vi "Reinitialize.vi"(8 "error in (no error)":errorcluster, 11 "ProPar in":refnum<class "PL Bronkhorst ProPar.lvclass">) -> (0 "error out":errorcluster, 3 "ProPar out":refnum<class "PL Bronkhorst ProPar.lvclass">)   [LabVIEW 2015, in "PL Bronkhorst ProPar.lvclass"]
doc: "Reinitializes connection to device based on previously specified settings."
uses:
  PL Bronkhorst ProPar.lvclass
  PL Bronkhorst ProPar.lvclass/PL Bronkhorst ProPar.ctl
  <vilib>/Instr/_visa.llb/VISA Configure Serial Port (Instr).vi
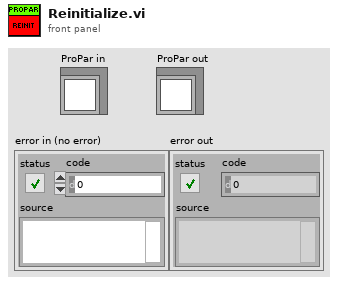
[diagram p1: front panel]
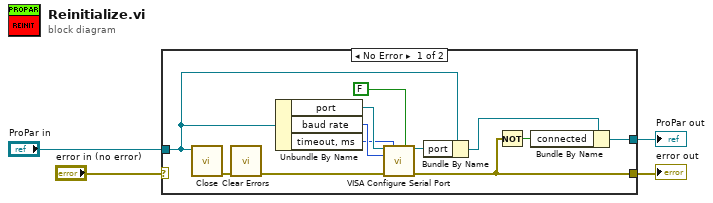
[diagram p0: block diagram]
diagram:
  n1 = case shown="No Error" "error in (no error)" {
    selector: "error in (no error)" -> [_ w17]
    tunnel: "ProPar in" -> [w16 w18]
    tunnel: [w13 w18] -> w3
    tunnel: [w9 w17] -> w2
    frame No Error {
      n2 = call "Close.vi"("ProPar in"=w16) -> ("error out"=w6:errorcluster)  [unwired: 10 in]
      n3 = call <vilib>:"Clear Errors.vi"("error in (no error)"=w6) -> ("error out"=w5:errorcluster)  [unwired: 5 in, 1 out]
      n4 = Unbundle By Name(w16) -> ("port"=w11:refnum<visa-resource-name>, "baud rate"=w12:u32, "timeout, ms"=w7:u32)
      n5 = call-poly "VISA Configure Serial Port"("VISA resource name"=w11, "timeout (10sec)"=w7, "Enable Termination\nChar (T)"=FALSE ("Enable Termination\nChar (T)"), "baud rate (9600)"=w12, "error in (no error)"=w5) -> ("VISA resource name out"=w10:refnum<visa-resource-name>, "error out"=w9:errorcluster)  [unwired: 9 in]
      n6 = Bundle By Name(cluster=w16, "port"=w10) -> (w15:refnum<class "PL Bronkhorst ProPar.lvclass">)
      n7 = Not(x=w9) -> (.not. x?=w14:bool)
      n8 = Bundle By Name(cluster=w15, "connected"=w14) -> (w13:refnum<class "PL Bronkhorst ProPar.lvclass">)
    }
    frame Error {
    }
  }
  "ProPar out" <- w3
  "error out" <- w2
